vi "ROI entry-Redraw mode logic.vi"(11 "Input cluster":T2 {"ROIs Info []"."FOV" min=1.0 max=10.0 step=1.0; "ROIs Info []"."Frame Size" min=1.0 max=10.0 step=1.0; "ROIs Info []"."Laser Power" min=1.0 max=10.0 step=0.10000000149011612; "ROIs Info []"."Rel. Resolution" min=1.0 max=10.0 step=1.0; "ROIs Info []"."POI Dwell time" min=1.0 max=10.0 step=0.10000000149011612; "ROIs Info []"."Zoom" min=1.0 max=10.0 step=0.10000000149011612; "Last Image Display Event info"."Tool" items=["None", "Selection Tool", "Point Tool", "Line Tool", "Rectangle Tool", "Oval Tool", "Polygon Tool", "ClosedFreehandTool", "Annulus Tool", "Rotated Rectangle Tool", "Zoom Tool", "Pan Tool", "Polyline Tool", "Freehand Tool"]; "Last Image Display Event info"."Type" items=["No Event"=0, "Click Event"=1, "Draw Event"=2, "Size Event"=4, "Scroll Event"=5, "Double Click Event"=8]}) -> (3 "Mode":T1)   [LabVIEW 2020]
uses:
  Typedefs/ROI Entry screen VI interface 1.ctl
  Typedefs/Last Image Display Event info.ctl
  Typedefs/ROI spec.ctl
  Typedefs/ROI ID Enum.ctl
  ROI Entry screen/Typedefs/Redraw ROI.ctl
  ROI Entry screen/Globals/gl_ROI Entry UI globals.vi
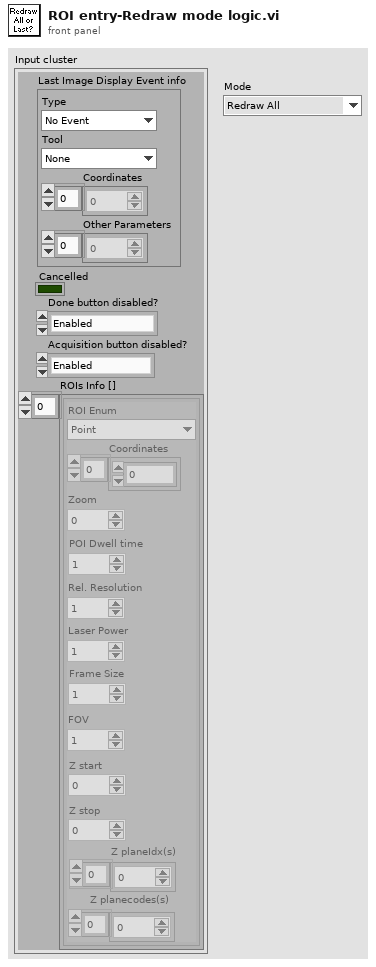
[diagram p1: front panel]
types:
  T1 = typedef "Redraw ROI.ctl" = enum16{"Redraw All", "Redraw Deselected", "Draw Last", "Redraw Selected"}
  T2 = typedef "ROI Entry screen VI interface 1.ctl" = cluster{"Last Image Display Event info":T3, "ROIs Info []":T4[], "Cancelled":bool, "Done button disabled?":enum8{"Enabled", "Disabled", "Disabled and Grayed Out"}, "Acquisition button disabled?":enum8{"Enabled", "Disabled", "Disabled and Grayed Out"}}
  T3 = typedef "Last Image Display Event info.ctl" = cluster{"Type":i32, "Tool":i32, "Coordinates":i32[], "Other Parameters":sgl[]}
  T4 = typedef "ROI spec.ctl" = cluster{"ROI Enum":T5, "Coordinates":i32[], "Zoom":dbl, "POI Dwell time":dbl, "Rel. Resolution":dbl, "Laser Power":dbl, "Frame Size":dbl, "FOV":dbl, "Z start":dbl, "Z stop":dbl, "Z planeIdx(s)":i32[], "Z planecodes(s)":u8[]}
  T5 = typedef "ROI ID Enum.ctl" = enum16{"Point", "MiniScan", "Comp. MiniScan", "Rectangle", "Comp. volume", "Arb. plane point", "None"}
  T6 = typedef "ROI entry screen ctrl refs cluster.ctl" = cluster{"Done button":refnum<vi>, "Imaging button":refnum<vi>, "Acquisition button":refnum<vi>, "Scan dwell time per pixel (us)":refnum<vi>, "# of planes":refnum<vi>, "Zoom Ctrl":refnum<vi>, "Equal size":refnum<vi>, "Channel":refnum<vi>, "Image Display":refnum<vi>, "Z-Plane Selector":refnum<vi>, "Number of lines left":refnum<vi>, "Z-stack folder path":refnum<vi>, "POI Density":refnum<vi>, "Arb Plane Entry":refnum<vi>, "Whole Plane":refnum<vi>, "Line Mode":refnum<vi>, "Clear Last":refnum<vi>, "Clear All":refnum<vi>, "Delete Lines":refnum<vi>, "Trial Length (sec)":refnum<vi>, "Palette Type":refnum<vi>, "Intensity slider":refnum<vi>, "# POI":refnum<vi>, "Max Z Proj":refnum<vi>, "Zplane ind":refnum<vi>, "Wavelength (nm)":refnum<vi>, "Number of Trials":refnum<vi>, "Funct stim.trig.enable":refnum<vi>, "Funct stim.trig.delay (s)":refnum<vi>, "Line Mode":refnum<vi>, "Step size (µm)":refnum<vi>, "ROI move mode":refnum<vi>, "Cool-down time (s)":refnum<vi>, "Enable cool-down time":refnum<vi>, "Motor Z ind. (um)":refnum<vi>, "AOL Z ind. (um)":refnum<vi>, "Load Reference Image":refnum<vi>, "Rel.  Res.":refnum<vi>, "ROI LIST":refnum<vi>, "Show All":refnum<vi>, "ROI Type":refnum<vi>, "Start Plane":refnum<vi>, "Stop Plane":refnum<vi>, "Offset ROI":refnum<vi>, "Tab Control":refnum<vi>, "Laser Power(%)":refnum<vi>, "Cycle rate":refnum<vi>, "FOV (Ind.)":refnum<vi>, "Frame Size (Ind.)":refnum<vi>, "Resolution (Ind.)":refnum<vi>, "Pixel Density (Ind)":refnum<vi>, "Laser Power (Ind.)":refnum<vi>, "Dwell Time (Ind.)":refnum<vi>, "Adj MC":refnum<vi>}
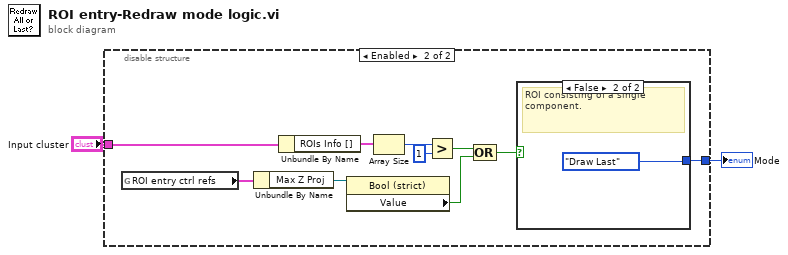
[diagram p0: block diagram]
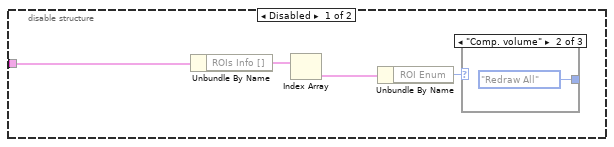
[diagram p2: hidden frame]
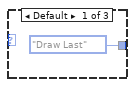
[diagram p3: hidden frame]
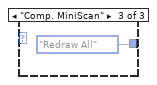
[diagram p4: hidden frame]
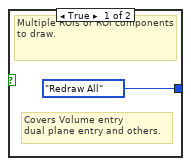
[diagram p5: hidden frame]
diagram:
  n1 = disable-structure shown="Enabled" {
    disable-tunnel: "Input cluster" -> [w6 w19]
    disable-tunnel: [_ w18] -> w1
    frame Disabled {
      n2 = Unbundle By Name(w6) -> ("ROIs Info []"=w5:T4[])
      n3 = Index Array(array=w5) -> (element=w3:T4)  [unwired: 1 in]
      n4 = Unbundle By Name(w3) -> ("ROI Enum"=w4:T5)
      n5 = case shown="\"Comp. volume\"" w4 {
        tunnel: [enum16{"Redraw All", "Draw Last"}."Draw Last" ("Mode") enum16{"Redraw All", "Draw Last"}."Redraw All" ("Mode") enum16{"Redraw All", "Draw Last"}."Redraw All" ("Mode")] -> _
        frame Default {
        }
        frame "Comp. volume" {
        }
        frame "Comp. MiniScan" {
        }
      }
    }
    frame Enabled {
      n6 = global read "gl_ROI Entry UI globals.vi" "ROI entry ctrl refs"() -> (w13:T6)
      n7 = Unbundle By Name(w13) -> ("Max Z Proj"=w14:refnum<vi>)
      n8 = Unbundle By Name(w19) -> ("ROIs Info []"=w17:T4[])
      n9 = property class="Bool (strict)"(reference=w14) -> ("Value"=w12:bool)  [unwired: 1 in, 2 out]
      n10 = Array Size(array=w17) -> (size(s)=w16:i32)
      n11 = Greater?(x=w16, y=1) -> (0:w11:bool)
      n12 = Compound Arithmetic op=OR(w11, w12) -> (w10:bool)
      n13 = case shown="False" w10 {
        tunnel: [Redraw_ROI."Redraw All" ("Mode") Redraw_ROI."Draw Last" ("Mode")] -> w18
        frame True {
          # "Covers Volume entry\ndual plane entry and others."
          # "Multiple ROIs or ROI components to draw."
        }
        frame False {
          # "ROI consisting of a single component."
        }
      }
    }
  }
  "Mode" <- w1
